vi "Read ESI Files on RT Target.vi"(8 "error in":errorcluster, 11 "Target IP":string) -> (0 "error out":errorcluster, 3 "Existing Target Profiles":string[](array[string]))   [LabVIEW 2020, in "SEECD System Explorer.lvlib"]
uses:
  SEECD System Explorer.lvlib
  <vilib>/FTP/NI_FTP.lvlib
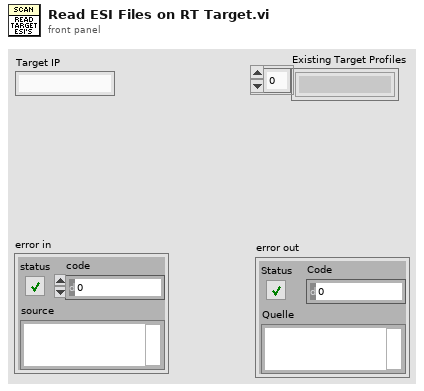
[diagram p1: front panel]
types:
  T1 = typedef "_fileTransferProtocol.ctl" = enum16{"Ftp", "WebDAV", "None"}
  T2 = typedef "_protocolSession.ctl" = cluster{"FTP session":T3, "WebDAV sssion":T4}
  T3 = typedef "NI_FTP.lvlib/FTP Session.ctl" = refnum<k5>
  T4 = typedef "NI_WebDAV.lvlib/SessionHandle.ctl" = refnum<k1>
  T5 = typedef "NI_FTP.lvlib/FTP File Info.ctl" = cluster{"type":enum16{"unknown", "file", "dir", "link"}, "permissions":string, "owner":string, "group":string, "size":i32, "date":string, "name":string, "link name":string}
  T6 = typedef "NI_WebDAV.lvlib/FileInfo.ctl" = cluster{"type":string, "size":u64, "last modification":timestamp, "display name":string, "uri":string}
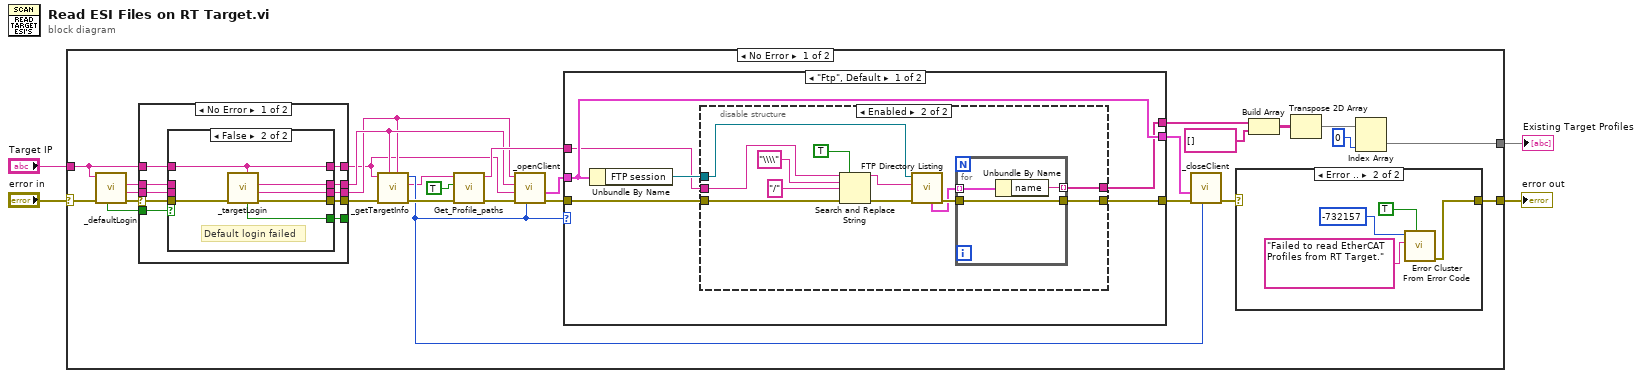
[diagram p0: block diagram]
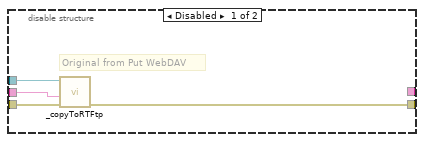
[diagram p5: hidden frame]
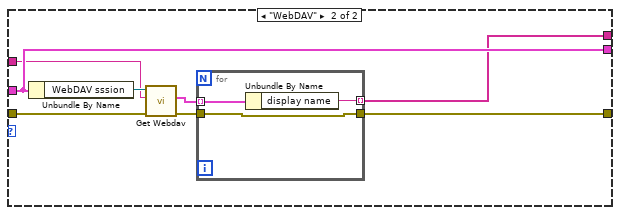
[diagram p6: hidden frame]
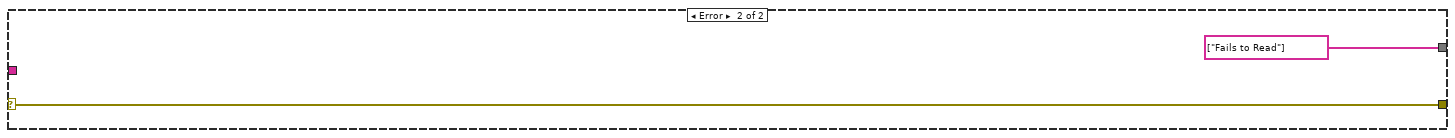
[diagram p7: hidden frame]
diagram:
  n1 = case shown="No Error" "error in" {
    selector: "error in" -> [w11 w96]
    tunnel: "Target IP" -> [w7 _]
    tunnel: [w5 w96] -> w2
    tunnel: [w29 string[] ["Fails to Read"]] -> w1
    frame No Error {
      n2 = call <resource>:"_defaultLogin.vi"("error in"=w11, "Target IP"=w7) -> ("error out"=w14:errorcluster, "password out"=w15:string, "user name out"=w16:string, "correct login?"=w13:bool)  [unwired: 6 in]
      n3 = case shown="No Error" w14 {
        selector: w14 -> [w41 w58]
        tunnel: [w47 _] -> w10
        tunnel: [w46 _] -> w9
        tunnel: [w45 _] -> _
        tunnel: [w44 w58] -> w12
        tunnel: w16 -> [w43 _]
        tunnel: w15 -> [w42 _]
        tunnel: w13 -> [w40 _]
        tunnel: w7 -> [w39 _]
        tunnel: [w38 _] -> w8
        frame No Error {
          n4 = case shown="False" w40 {
            tunnel: [w51 w57] -> w47
            tunnel: [w50 w56] -> w46
            tunnel: [w49 w55] -> w44
            tunnel: [_ w52] -> w45
            tunnel: w43 -> [w51 _]
            tunnel: w42 -> [w50 _]
            tunnel: w41 -> [w49 w54]
            tunnel: w39 -> [w48 w53]
            tunnel: [w48 w53] -> w38
            frame True {
            }
            frame False {
              # "Default login failed"
              n5 = call <resource>:"_targetLogin.vi"("Target IP"=w53, "error in"=w54) -> ("error out"=w55:errorcluster, "Password out"=w56:string, "Username out"=w57:string, "cancel?"=w52:bool)  [unwired: 6 in]
            }
          }
        }
        frame Error {
        }
      }
      n6 = call <resource>:"_getTargetInfo.vi"("password"=w9, "user name"=w10, "error in"=w12, "Target IP"=w8) -> ("error out"=w32:errorcluster, "Target OS"=w30:string, "protocol"=w31:T1)  [unwired: 4 in, 1 out]
      n7 = call "Get_Profile_paths.vi"("error in (no error)"=w32, "Target?"=TRUE, "OSArch"=w30) -> ("error out"=w28:errorcluster, "profileDestPath"=w27:string)  [unwired: 7 in]
      n8 = call <resource>:"_openClient.vi"("protocol"=w31, "error in (no error)"=w28, "Target IP"=w8, "user name"=w10, "password"=w9) -> ("error out"=w17:errorcluster, "Cluster"=w20:T2)  [unwired: 5 in]
      n9 = case shown="\"Ftp\", Default" w31 {
        tunnel: w20 -> [w62 w89]
        tunnel: [w61 w86] -> w18
        tunnel: w17 -> [w64 w90]
        tunnel: [w62 w89] -> w19
        tunnel: w27 -> [w60 w88]
        tunnel: [w59 w84] -> w24
        frame "Ftp", Default {
          n10 = Unbundle By Name(w62) -> ("FTP session"=w63:T3)
          n11 = disable-structure shown="Enabled" {
            disable-tunnel: w64 -> [w68 w77]
            disable-tunnel: w63 -> [w67 w75]
            disable-tunnel: [w66 w72] -> w61
            disable-tunnel: w60 -> [w65 w78]
            disable-tunnel: [_ w71] -> w59
            frame Disabled {
              # "Original from Put WebDAV"
              n12 = call <resource>:"_copyToRTFtp.vi"("error in (no error)"=w68, "directory path"=w65, "TCP Network Connection in"=w67) -> ("error out"=w66:errorcluster)  [unwired: 7 in, 1 out]
            }
            frame Enabled {
              n13 = Search and Replace String(replace all?=TRUE ("replace all? (F)"), input string=w78, search string="\\\\", replace string="/" ("replace string (\"\")"), error in=w77) -> (result string=w74:string, error out=w76:errorcluster)  [unwired: 3 in, 2 out]
              n14 = call <vilib>:"FTP Directory Listing.vi"("error in (no error)"=w76, "directory path"=w74, "ftp session"=w75) -> ("error out"=w73:errorcluster, "dir list"=w70:T5[])  [unwired: 4 in, 3 out]
              n15 = for {
                tunnel: w73 -> [w83]
                tunnel: [w83] -> w72
                tunnel: w70 -> [w82] mode=indexing
                tunnel: [w81] -> w71 mode=indexing
                n16 = Unbundle By Name(w82) -> ("name"=w81:string)
              }
            }
          }
        }
        frame "WebDAV" {
          n17 = Unbundle By Name(w89) -> ("WebDAV sssion"=w91:T4)
          n18 = call "Get Webdav.vi"("error in (no error)"=w90, "relative uri"=w88, "Refnum in"=w91) -> ("error out"=w87:errorcluster, "file list"=w85:T6[])  [unwired: 6 in, 1 out]
          n19 = for {
            tunnel: w87 -> [w94]
            tunnel: [w94] -> w86
            tunnel: w85 -> [w93] mode=indexing
            tunnel: [w92] -> w84 mode=indexing
            n20 = Unbundle By Name(w93) -> ("display name"=w92:string)
          }
        }
      }
      n21 = call <resource>:"_closeClient.vi"("protocol"=w31, "error in"=w18, "session in"=w19) -> ("error out"=w6:errorcluster)  [unwired: 8 in]
      n22 = case shown="Error .." w6 {
        selector: w6 -> [w33 _]
        tunnel: [w33 w34] -> w5
        frame No Error {
        }
        frame Error {
          n23 = call <vilib>:"Error Cluster From Error Code.vi"("show call chain? (False)"=TRUE, "error message (\"\")"="Failed to read EtherCAT Profiles from RT Target." ("source"), "error code (0)"=-732157 ("code")) -> ("error out"=w34:errorcluster)  [unwired: 6 in]
        }
      }
      n24 = Build Array(w24, string[] [] ("Element")) -> (w26:string[][])
      n25 = Transpose 2D Array(2D array=w26) -> (transposed array=w23:string[][])
      n26 = Index Array(array=w23, index (col)=0) -> (element=w29:string[])  [unwired: 1 in]
    }
    frame Error {
    }
  }
  "error out" <- w2
  "Existing Target Profiles" <- w1
